vi "Armstrong Number Check.vi"() -> ()   [LabVIEW 2026]
panel:
  out "Status":string
  in  "Input Number(N)":dbl
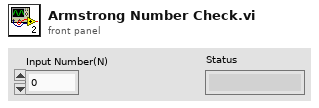
[diagram p1: front panel]
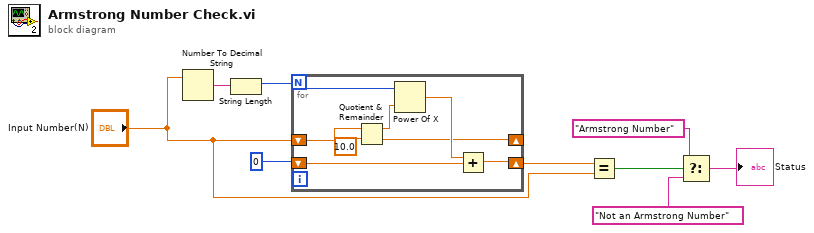
[diagram p0: block diagram]
diagram:
  n1 = Number To Decimal String(number="Input Number(N)") -> (decimal integer string=w9:string)  [unwired: 1 in]
  n2 = String Length(string=w9) -> (length=w7:i32)
  n3 = for {
    N: w7 -> [w11]
    shift-right: [w10] -> _
    shift-left: "Input Number(N)" -> [w17]
    shift-right: [w12] -> w6
    shift-left: 0 -> [w14]
    n4 = Quotient & Remainder(x=w17, y=10.0) -> (x-y*floor(x/y)=w15:dbl, floor(x/y)=w10:dbl)
    n5 = Power Of X(1:w15, 2:w11) -> (0:w13:dbl)
    n6 = Add(x=w13, y=w14) -> (x+y=w12:dbl)
  }
  n7 = Equal?(x=w6, y="Input Number(N)") -> (x = y?=w4:bool)
  n8 = Select(t="Armstrong Number", s=w4, f="Not an Armstrong Number") -> (s? t:f=→"Status":string)
